vi "Add Link Button.vi"(8 "error in (no error)":errorcluster, 9 "URl":string, 10 "Content":string, 11 "ToastBuilder in":refnum<class "ToastBuilder.lvclass">) -> (0 "error out":errorcluster, 3 "ToastBuilder out":refnum<class "ToastBuilder.lvclass">)   [LabVIEW 2026, in "ToastNotification.lvlib" / "ToastBuilder.lvclass"]
doc: "Adds a link button to the current toast using the encapsulated native builder. Content is the visible button text and URl is the URI string opened by Windows when the button is clicked. Create the builder before calling this method, then show the toast separately. The button uses Protocol activation; this button click does not invoke ActivationHandler.Handle Activation. Clicking the toast body is a separate activation. An incoming error passes the class and error through unchanged. The method does not close the builder or expose .NET references; its owner must call Close after the last use. URL validation and native errors are delegated to the toolkit and Windows."
uses:
  ToastBuilder.lvclass
  ToastBuilder.lvclass/ToastBuilder.ctl
  Read Builder Reference.vi
  Write Builder Reference.vi
  Toast Native/Toast Native.lvlib
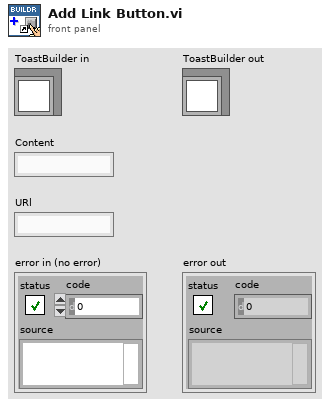
[diagram p1: front panel]
types:
  T1 = typedef "ToastNotification.lvlib/ToastBuilder.lvclass/Builder Reference.ctl" = refnum<k24>
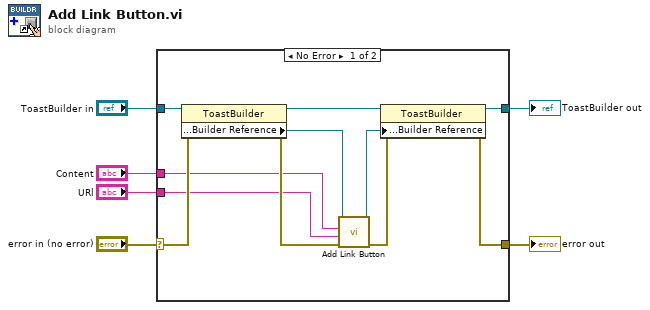
[diagram p0: block diagram]
diagram:
  n1 = case shown="No Error" "error in (no error)" {
    selector: "error in (no error)" -> [w15 w19]
    tunnel: [w13 w19] -> w5
    tunnel: [w14 w18] -> w3
    tunnel: "ToastBuilder in" -> [w17 w18]
    tunnel: "Content" -> [w8 _]
    tunnel: "URl" -> [w7 _]
    frame No Error {
      n2 = property class="ToastBuilder"(reference=w17, error in=w15) -> (reference out=w16:refnum<class "ToastBuilder.lvclass">, error out=w12:errorcluster, "Public:Properties:Builder Reference"=w10:T1)
      n3 = call "Add Link Button.vi"("error in (no error)"=w12, "URl"=w7, "content"=w8, "reference"=w10) -> ("error out"=w11:errorcluster, "reference out"=w9:refnum<k24>)  [unwired: 6 in]
      n4 = property class="ToastBuilder"(reference=w16, error in=w11, "Public:Properties:Builder Reference"=w9) -> (reference out=w14:refnum<class "ToastBuilder.lvclass">, error out=w13:errorcluster)
    }
    frame Error {
    }
  }
  "error out" <- w5
  "ToastBuilder out" <- w3
